vi "update asset metadata.vi"(9 "property key-value pairs":cluster{"key":string, "value":string}[](array[cluster]), 10 "Labels":string[](array[string]), 11 "asset":refnum<class "asset.lvclass">) -> (0 "error out":errorcluster, 3 "updated asset":refnum<class "asset.lvclass">)   [LabVIEW 2020, in "nominal core steps.lvlib"]
doc: "Update an asset obtained with `create asset` or `get asset` with properties and labels.\n<b> </b> <b> </b>"
uses:
  nominal core steps.lvlib
  <vilib>/Nominal/Nominal IO Client/lv_src/asset/asset.lvclass
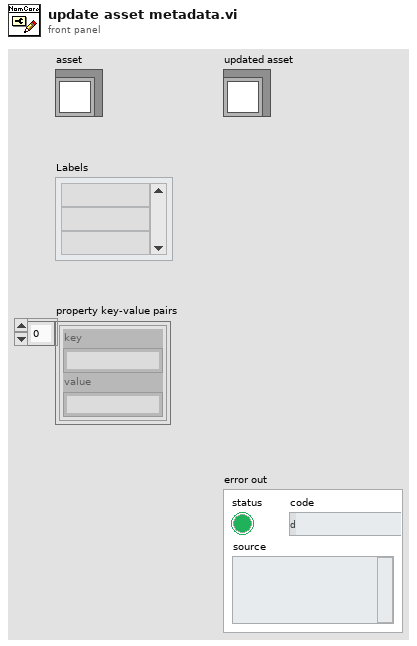
[diagram p1: front panel]
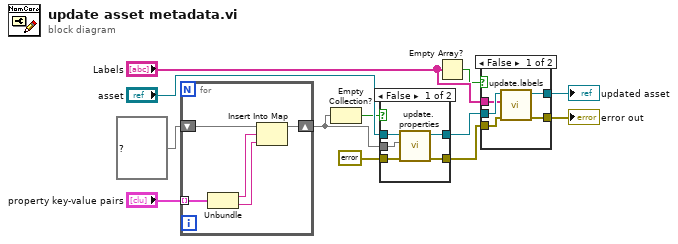
[diagram p0: block diagram]
diagram:
  n1 = for {
    tunnel: "property key-value pairs" -> [w17] mode=indexing
    shift-right: [w14] -> w1
    shift-left: map{string, string} {} ("map") -> [w15]
    n2 = Unbundle(w17) -> ("key"=w16:string, "value"=w13:string)
    n3 = Insert Into Map(map in=w15, key=w16, value=w13) -> (map out=w14:map{string, string})  [unwired: 2 out]
  }
  n4 = Empty Collection?(1:w1) -> (0:w3:bool)
  n5 = case shown="False" w3 {
    tunnel: [w22 w24] -> w12
    tunnel: [w21 w23] -> w11
    tunnel: "asset" -> [w20 w24]
    tunnel: w1 -> [w18 _]
    tunnel: errorcluster {"status"=FALSE, "code"=0, "source"=""} ("error in") -> [w19 w23]
    frame False {
      n6 = call <vilib>:"update.properties.vi"("error in"=w19, "Properties"=w18, "asset in"=w20) -> ("error out"=w21:errorcluster, "asset out"=w22:refnum<class "asset.lvclass">)  [unwired: 7 in]
    }
    frame True {
    }
  }
  n7 = Empty Array?(array="Labels") -> (empty?=w6:bool)
  n8 = case shown="False" w6 {
    tunnel: w12 -> [w29 w31]
    tunnel: w11 -> [w28 w30]
    tunnel: [w27 w31] -> w10
    tunnel: [w26 w30] -> w9
    tunnel: "Labels" -> [w25 _]
    frame False {
      n9 = call <vilib>:"update.labels.vi"("error in"=w28, "Labels"=w25, "asset in"=w29) -> ("error out"=w26:errorcluster, "asset out"=w27:refnum<class "asset.lvclass">)  [unwired: 7 in]
    }
    frame True {
    }
  }
  "updated asset" <- w10
  "error out" <- w9
